vi "Connect_direct (Dynamic).vi"(7 "ORMDriver":string(combo)="pgsql_jdp", 8 "error in (no error)":errorcluster, 11 "Connection String":string) -> (0 "error out":errorcluster, 3 "SqlMapper out":refnum<class "SqlMapper.lvclass">)   [LabVIEW 2020, in "ORM_API_jdp.lvlib"]
uses:
  ORM_API_jdp.lvlib
  <vilib>/Viviota/shared/ORM.lvlibp/SqlMapper/SqlMapper.lvclass
  <vilib>/Viviota/shared/ORM.lvlibp/DbConnection/DbConnection.lvclass
  <vilib>/Utility/LVLibp/NI_PackedLibraryUtility.lvlib
panel:
  # "to add quotes to SQLite table names\ninclude:\n\nORMQuotesOnTableName=true|false;"
  # "postgresql: host=localhost port=5432 dbname=mydb\n(accepts spaces or ; as delmiter)\n\nsqlite: Data Source=C:\\Users\\Public\\Documents\\test.db"
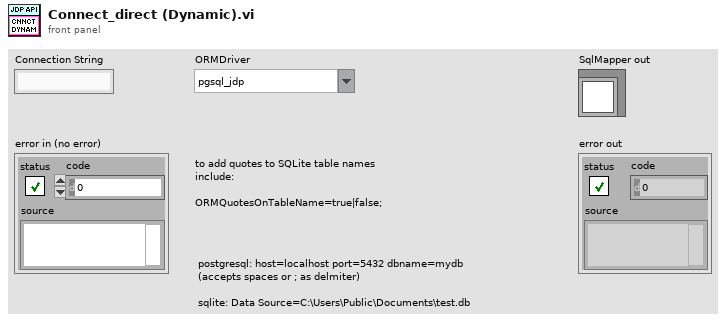
[diagram p1: front panel]
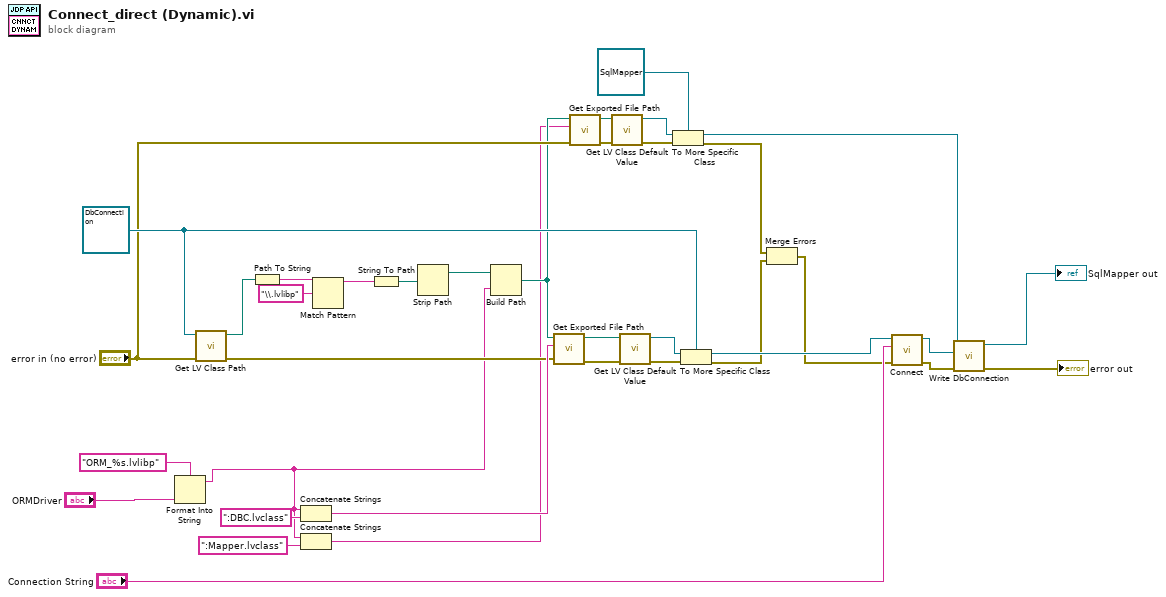
[diagram p0: block diagram]
diagram:
  w20 = refnum<class "DbConnection.lvclass"> refnum ("Dapper.lvlib:DbConnection.lvclass")
  n1 = Format Into String(format string="ORM_%s.lvlibp", "ORMDriver") -> (resulting string=w4:string)  [unwired: 2 in, 1 out]
  n2 = call <vilib>:"Get LV Class Path.vi"("error in (no error)"="error in (no error)", "object"=w20) -> ("error out"=w25:errorcluster, "class path"=w33:path)  [unwired: 8 in]
  n3 = Path To String(path=w33) -> (string=w32:string)
  n4 = Concatenate Strings(w4, ":DBC.lvclass" ("string")) -> (w26:string)
  n5 = Concatenate Strings(w4, ":Mapper.lvclass" ("string")) -> (w1:string)
  n6 = Match Pattern(string=w32, regular expression="\\.lvlibp") -> (before substring=w30:string)  [unwired: 1 in, 3 out]
  n7 = String To Path(string=w30) -> (path=w29:path)
  n8 = Strip Path(path=w29) -> (stripped path=w27:path)  [unwired: 1 out]
  n9 = Build Path(base path=w27, name or relative path=w4) -> (appended path=w2:path)
  n10 = call <vilib>:"Get Exported File Path.vi"("error in (no error)"=w25, "qualified name"=w26, "packed library path"=w2) -> ("error out"=w24:errorcluster, "path"=w22:path)  [unwired: 7 in]
  n11 = call <vilib>:"Get Exported File Path.vi"("error in (no error)"="error in (no error)", "qualified name"=w1, "packed library path"=w2) -> ("error out"=w13:errorcluster, "path"=w15:path)  [unwired: 7 in]
  n12 = call <vilib>:"Get LV Class Default Value.vi"("error in (no error)"=w13, "class path"=w15) -> ("error out"=w14:errorcluster, "object"=w16:refnum<class>)  [unwired: 8 in]
  n13 = call <vilib>:"Get LV Class Default Value.vi"("error in (no error)"=w24, "class path"=w22) -> ("error out"=w23:errorcluster, "object"=w21:refnum<class>)  [unwired: 8 in]
  n14 = To More Specific Class(target class=refnum<class "SqlMapper.lvclass"> refnum ("Type In"), reference=w16, error in=w14) -> (specific class reference=w10:refnum<class "SqlMapper.lvclass">, error out=w9:errorcluster)
  n15 = To More Specific Class(target class=w20, reference=w21, error in=w23) -> (specific class reference=w19:refnum<class "DbConnection.lvclass">, error out=w8:errorcluster)
  n16 = Merge Errors(w9, w8) -> (w7:errorcluster)
  n17 = call-dynamic "Connect.vi"("error in (no error)"=w7, "Connection String"="Connection String", "DbConnection Type"=w19) -> ("error out"=w18:errorcluster, "DbConnection out"=w34:refnum<class "DbConnection.lvclass">)  [unwired: 7 in]
  n18 = call <vilib>:"Write DbConnection.vi"("error in (no error)"=w18, "Dapper.lvlib:DbConnection.lvclass"=w34, "SqlMapper in"=w10) -> ("error out"=→"error out":errorcluster, "SqlMapper out"=→"SqlMapper out":refnum<class "SqlMapper.lvclass">)  [unwired: 7 in]
